vi "get helper loop state.vi"() -> (3 "running":bool)   [LabVIEW 2018, in "XButton.lvlib" / "button3.xctl"]
uses:
  button3.xctl
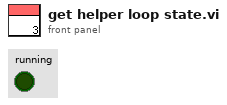
[diagram p1: front panel]
types:
  T1 = enum32{"Bad", "Idle", "Run top level", "Running"}
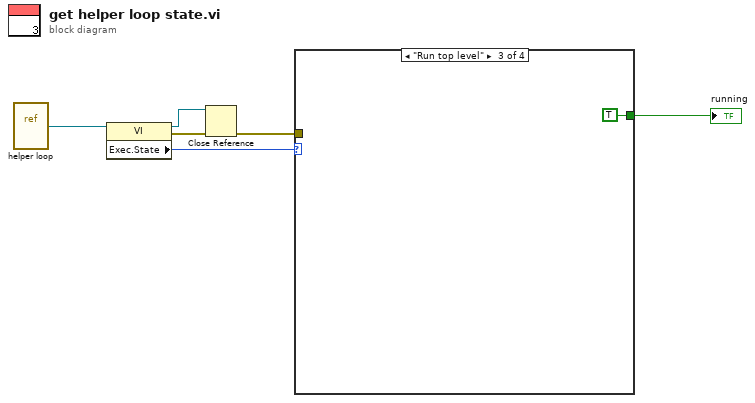
[diagram p0: block diagram]
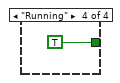
[diagram p4: hidden frame]
diagram:
  n1 = vi-ref "helper loop.vi"() -> (w6:refnum<vi>)
  n2 = property class="VI"(reference=w6) -> (reference out=w3:refnum<vi>, error out=w2:errorcluster, "Exec.State"=w5:T1)  [unwired: 1 in]
  n3 = Close Reference(reference=w3, error in (no error)=w2) -> (error out=w1:errorcluster)
  n4 = case shown="\"Run top level\"" w5 {
    tunnel: [_ _ TRUE TRUE] -> w4
    tunnel: w1 -> [_ _ _ _]
    frame "Bad", Default {
    }
    frame "Idle" {
    }
    frame "Run top level" {
    }
    frame "Running" {
    }
  }
  "running" <- w4
